vi "Read Register.vi"() -> ()   [LabVIEW 2020]
uses:
  g_industrial_cam/Camera/Camera.lvclass/Camera.ctl
  g_industrial_cam/Camera/GetSetRegister.vi
  g_industrial_cam/Camera/Check Not Disconnected.vi
  <vilib>/Utility/error.llb/Error Cluster From Error Code.vi
  g_industrial_cam/Camera/Camera.lvclass
panel:
  out "Pixel Dyamic Range Max":string
  out "Device User ID":string
  out "error out":errorcluster
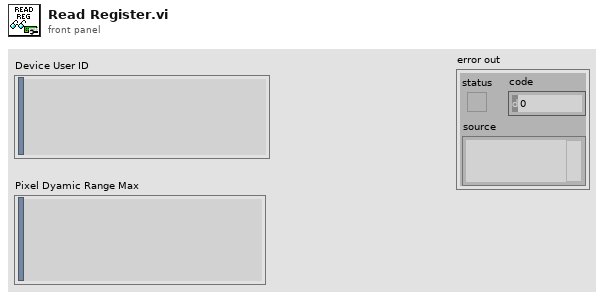
[diagram p1: front panel]
types:
  T1 = typedef "Device Enumeration.ctl" = cluster{"ID":string, "Protocol":string, "Vendor":string, "Model":string, "Serial":string, "Address":string}
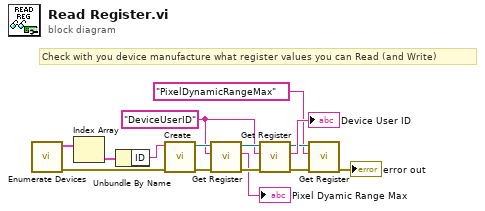
[diagram p0: block diagram]
diagram:
  w7 = "DeviceUserID" ("Register Name")
  # "Check with you device manufacture what register values you can Read (and Write)"
  n1 = call "Enumerate Devices.vi"() -> ("error out"=w13:errorcluster, "Devices"=w15:T1[])  [unwired: 10 in]
  n2 = Index Array(array=w15) -> (element=w14:T1)  [unwired: 1 in]
  n3 = Unbundle By Name(w14) -> ("ID"=w12:string)
  n4 = call "Create.vi"("error in (no error)"=w13, "Identifier (ID, IP etc)"=w12) -> ("error out"=w10:errorcluster, "Camera"=w11:refnum<class "Camera.lvclass">)  [unwired: 8 in]
  n5 = call "Get Register.vi"("error in (no error)"=w10, "Feature Name"=w7, "Camera in"=w11) -> ("error out"=w8:errorcluster, "Bytes Out"=→"Pixel Dyamic Range Max":string, "Camera"=w9:refnum<class "Camera.lvclass">)  [unwired: 6 in]
  n6 = call "Get Register.vi"("error in (no error)"=w8, "Feature Name"=w7, "Camera in"=w9) -> ("error out"=w4:errorcluster, "Bytes Out"=→"Device User ID":string, "Camera"=w5:refnum<class "Camera.lvclass">)  [unwired: 6 in]
  n7 = call "Get Register.vi"("error in (no error)"=w4, "Feature Name"="PixelDynamicRangeMax", "Camera in"=w5) -> ("error out"=→"error out":errorcluster)  [unwired: 6 in, 2 out]
